vi "NR Change Modulation Status.vi"(8 "error in (no error)":errorcluster caption="에러 입력(에러 없음)", 10 "Modulation":T1, 11 "Instrument Manager 입력":refnum<class "Instrument Manager.lvclass">) -> (0 "error out":errorcluster caption="에러 출력", 3 "Instrument Manager 출력":refnum<class "Instrument Manager.lvclass">)   [LabVIEW 2023, in "Instrument Manager.lvclass"]
uses:
  Instrument Manager.lvclass
  Instrument Manager.lvclass/Instrument Manager.ctl
  Module/ANRITSU Call Box/Type Definition/NR Modulation Type.ctl
  Module/ANRITSU Call Box/ANRITSU Call Box.lvlib
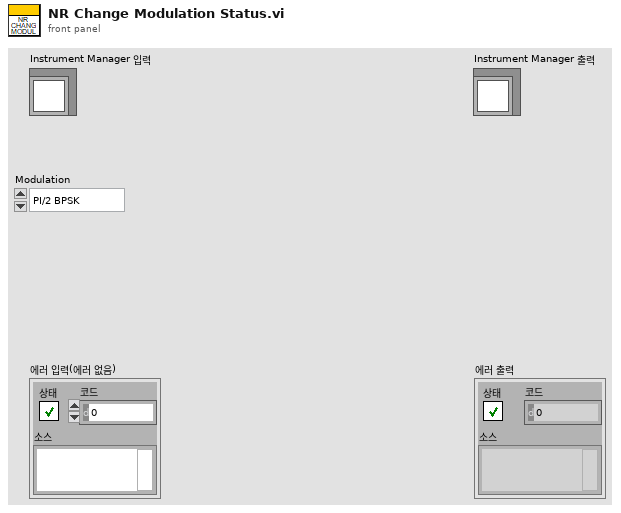
[diagram p1: front panel]
types:
  T1 = typedef "ANRITSU Call Box.lvlib/NR Modulation Type.ctl" = enum16{"PI/2 BPSK", "QPSK", "16QAM", "64QAM", "256QAM"}
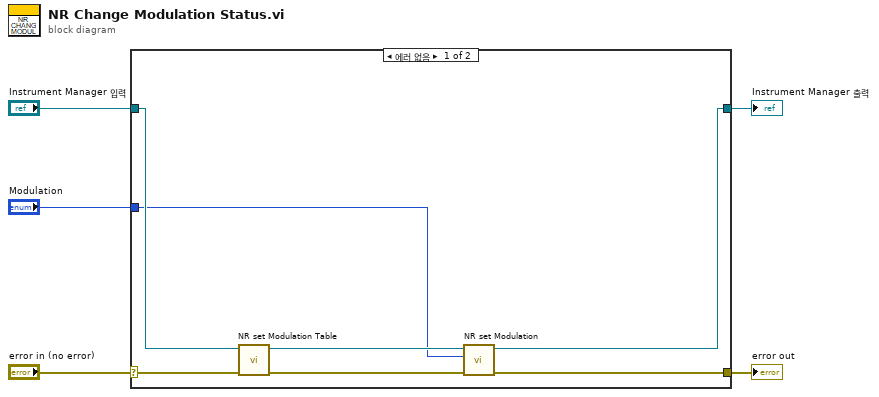
[diagram p0: block diagram]
diagram:
  n1 = case shown="에러 없음" "error in (no error)" {
    selector: "error in (no error)" -> [w12 w14]
    tunnel: [w10 w14] -> w4
    tunnel: [w7 w13] -> w2
    tunnel: "Instrument Manager 입력" -> [w9 w13]
    tunnel: "Modulation" -> [w6 _]
    frame No Error {
      n2 = call "NR set Modulation Table.vi"("error in (no error)"=w12, "Instrument Manager 입력"=w9) -> ("error out"=w11:errorcluster, "Instrument Manager 출력"=w8:refnum<class "Instrument Manager.lvclass">)  [unwired: 8 in]
      n3 = call "NR set Modulation.vi"("error in (no error)"=w11, "Modulation"=w6, "Instrument Manager 입력"=w8) -> ("error out"=w10:errorcluster, "Instrument Manager 출력"=w7:refnum<class "Instrument Manager.lvclass">)  [unwired: 7 in]
    }
    frame Error {
    }
  }
  "error out" <- w4
  "Instrument Manager 출력" <- w2
